vi "Dialog Tester - Preempt.vi"() -> ()   [LabVIEW 2021]
doc: "<b>TEST VI</b> checking the pre-empt action for pop up types"
uses:
  Standard/Input (DBL)/Input (DBL).lvclass
  Standard/Input (I32)/Input (I32).lvclass
  Standard/Input (String)/Input (String).lvclass
  Standard/Timeout/Timeout.lvclass
  Standard/Timeout One Button/Timeout One Button.lvclass
  Standard/Timeout Two Button/Timeout Two Button.lvclass
  Standard/Two Button/Two Button.lvclass
  Popup/Popup.lvclass
panel:
  out "Two-Button T.O. Choice? - val":bool
  out "Two-Button Choice? - val":bool
  out "Input Value (String - val)":string
  out "Input Value (I32 - val)":i32
  out "Input Value (DBL - close)":dbl
  out "Two-Button T.O. Choice? - close":bool
  out "Two-Button Choice? - close":bool
  out "Input Value (String - close)":string
  out "Input Value (I32 - close)":i32
  out "Input Value (DBL - val)":dbl
  out "iteration":i32
  in  "Error In":errorcluster
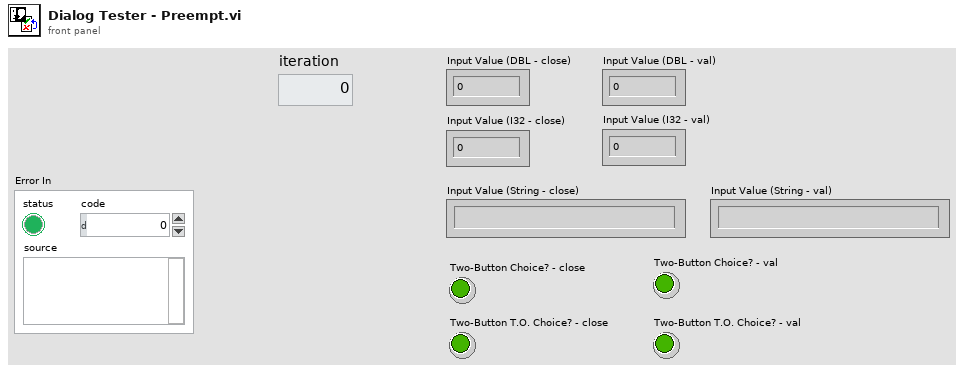
[diagram p1: front panel]
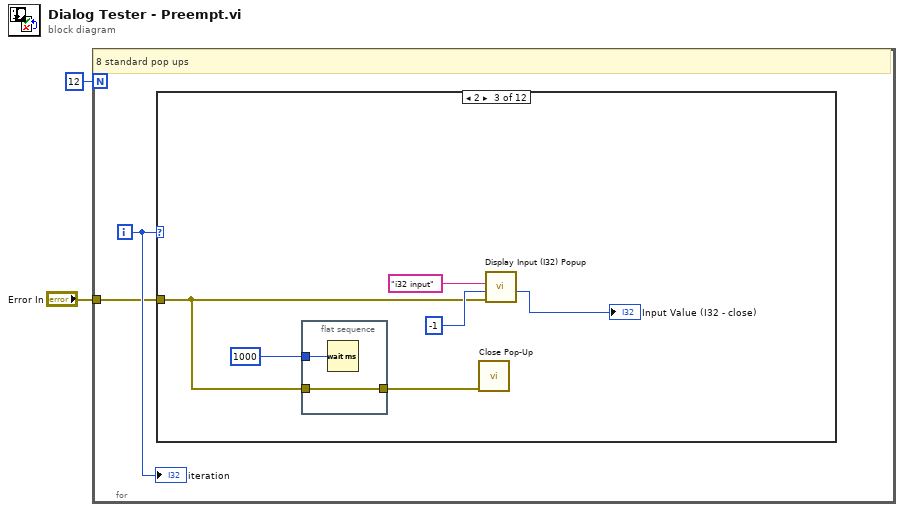
[diagram p0: block diagram]
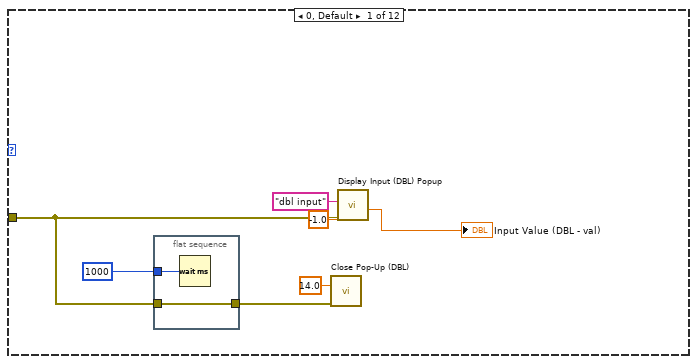
[diagram p2: hidden frame]
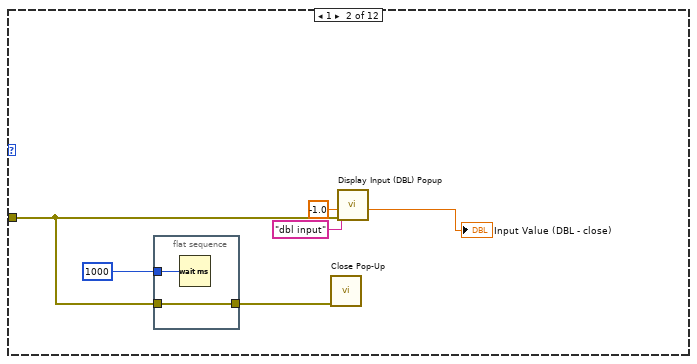
[diagram p3: hidden frame]
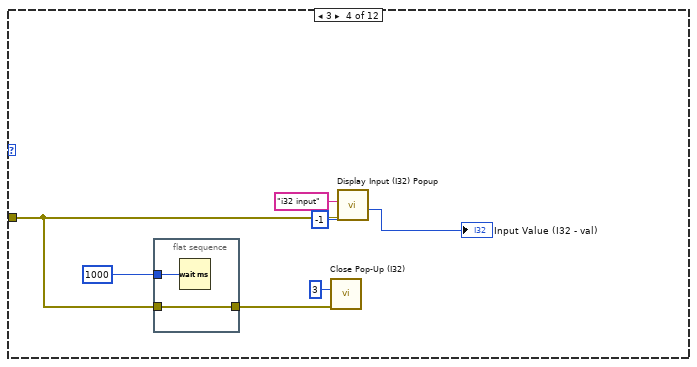
[diagram p4: hidden frame]
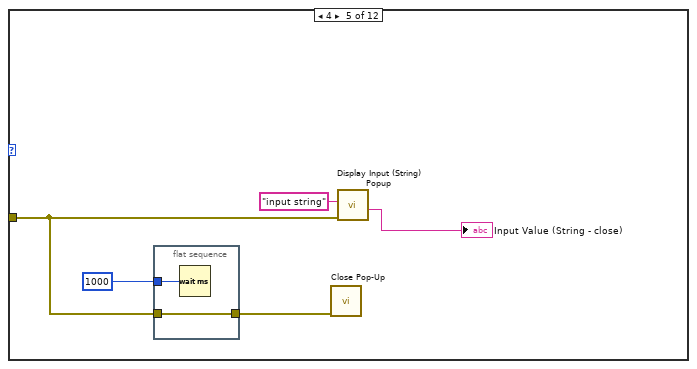
[diagram p5: hidden frame]
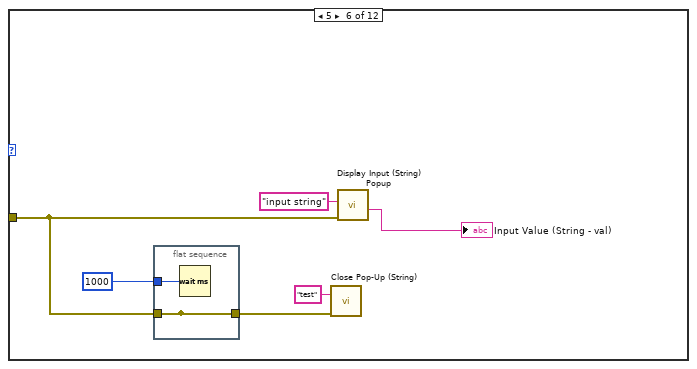
[diagram p6: hidden frame]
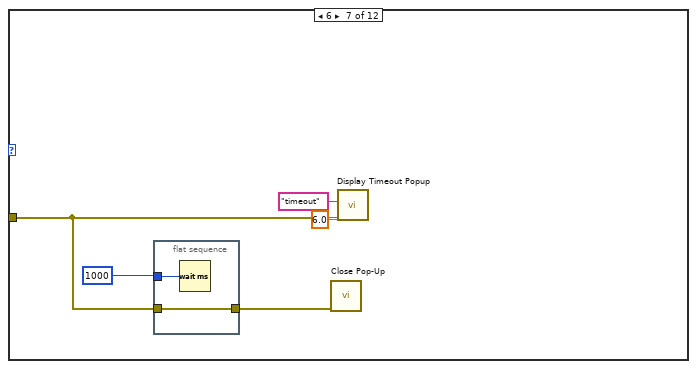
[diagram p7: hidden frame]
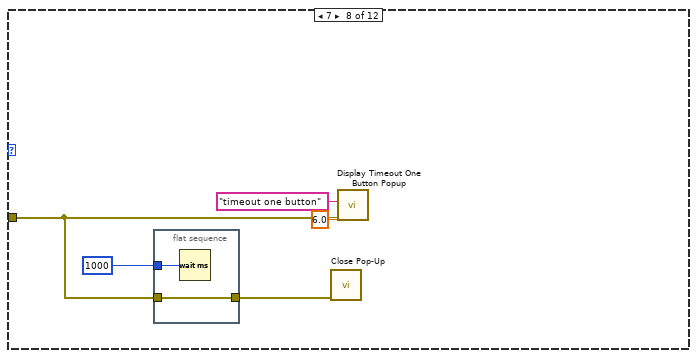
[diagram p8: hidden frame]
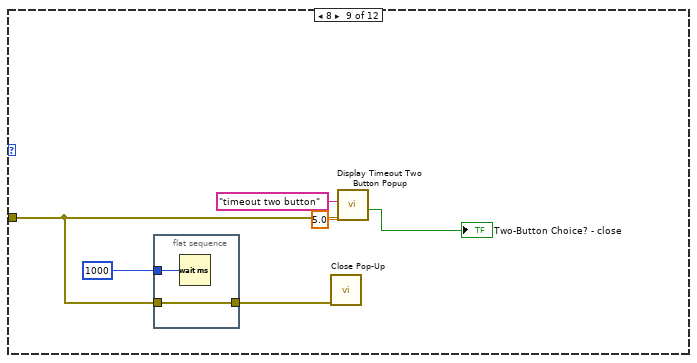
[diagram p9: hidden frame]
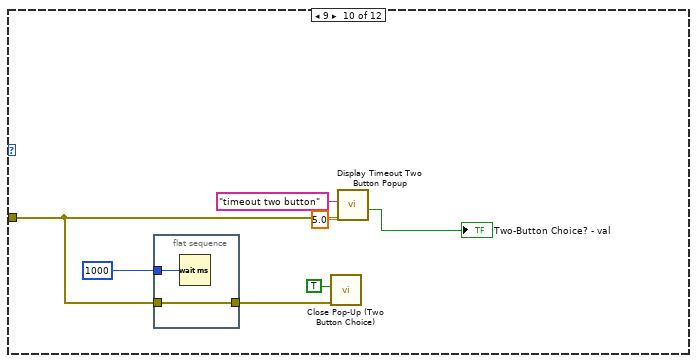
[diagram p10: hidden frame]
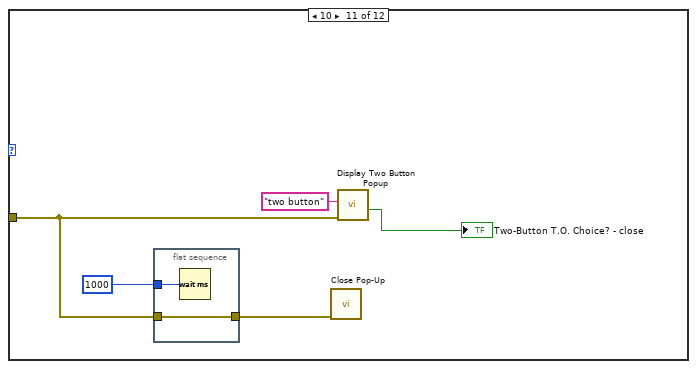
[diagram p11: hidden frame]
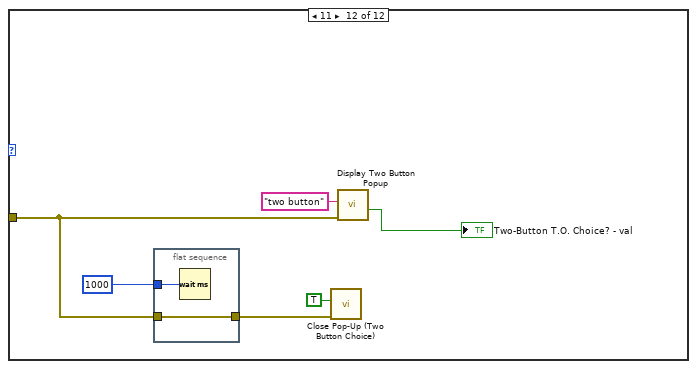
[diagram p12: hidden frame]
diagram:
  n1 = for {
    N: 12 -> [_]
    tunnel: "Error In" -> [w3]
    i -> [w4]
    # "8 standard pop ups"
    n2 = case shown="2" w4 {
      tunnel: w3 -> [w7 w16 w23 w31 w40 w47 w54 w62 w69 w77 w86 w93]
      frame 0, Default {
        n3 = flat-sequence {
          tunnel: u32 1000 ("milliseconds to wait") -> [w13]
          tunnel: [w12] -> w6
          tunnel: w7 -> [w12]
          frame #0 {
            n4 = Wait (ms)(milliseconds to wait=w13) -> ()  [unwired: 1 out]
          }
        }
        n5 = call "Close Pop-Up (DBL).vi"("error in"=w6, "DBL Default"=14.0) -> ()  [unwired: 9 in, 1 out]
        n6 = call "Display Input (DBL) Popup.vi"("error in"=w7, "Default Input"=-1.0, "Message"="dbl input") -> ("Input Value"=→"Input Value (DBL - val)":dbl)  [unwired: 7 in, 1 out]
      }
      frame 1 {
        n7 = flat-sequence {
          tunnel: u32 1000 ("milliseconds to wait") -> [w21]
          tunnel: [w20] -> w15
          tunnel: w16 -> [w20]
          frame #0 {
            n8 = Wait (ms)(milliseconds to wait=w21) -> ()  [unwired: 1 out]
          }
        }
        n9 = call "Close Pop-Up.vi"("error in"=w15) -> ()  [unwired: 10 in, 1 out]
        n10 = call "Display Input (DBL) Popup.vi"("error in"=w16, "Default Input"=-1.0, "Message"="dbl input") -> ("Input Value"=→"Input Value (DBL - close)":dbl)  [unwired: 7 in, 1 out]
      }
      frame 2 {
        n11 = flat-sequence {
          tunnel: u32 1000 ("milliseconds to wait") -> [w29]
          tunnel: [w28] -> w24
          tunnel: w23 -> [w28]
          frame #0 {
            n12 = Wait (ms)(milliseconds to wait=w29) -> ()  [unwired: 1 out]
          }
        }
        n13 = call "Close Pop-Up.vi"("error in"=w24) -> ()  [unwired: 10 in, 1 out]
        n14 = call "Display Input (I32) Popup.vi"("error in"=w23, "Default Input"=-1, "Message"="i32 input") -> ("Input Value"=→"Input Value (I32 - close)":i32)  [unwired: 7 in, 1 out]
      }
      frame 3 {
        n15 = flat-sequence {
          tunnel: u32 1000 ("milliseconds to wait") -> [w37]
          tunnel: [w36] -> _
          tunnel: w31 -> [w36]
          frame #0 {
            n16 = Wait (ms)(milliseconds to wait=w37) -> ()  [unwired: 1 out]
          }
        }
        n17 = call "Close Pop-Up (I32).vi"("error in"=w31, "I32 Default"=3) -> ()  [unwired: 9 in, 1 out]
        n18 = call "Display Input (I32) Popup.vi"("error in"=w31, "Default Input"=-1, "Message"="i32 input") -> ("Input Value"=→"Input Value (I32 - val)":i32)  [unwired: 7 in, 1 out]
      }
      frame 4 {
        n19 = flat-sequence {
          tunnel: u32 1000 ("milliseconds to wait") -> [w44]
          tunnel: [w43] -> w39
          tunnel: w40 -> [w43]
          frame #0 {
            n20 = Wait (ms)(milliseconds to wait=w44) -> ()  [unwired: 1 out]
          }
        }
        n21 = call "Close Pop-Up.vi"("error in"=w39) -> ()  [unwired: 10 in, 1 out]
        n22 = call "Display Input (String) Popup.vi"("error in"=w40, "Message"="input string") -> ("Input Value"=→"Input Value (String - close)":string)  [unwired: 8 in, 1 out]
      }
      frame 5 {
        n23 = flat-sequence {
          tunnel: u32 1000 ("milliseconds to wait") -> [w52]
          tunnel: [w51] -> w45
          tunnel: [w51] -> _
          tunnel: w47 -> [w51]
          frame #0 {
            n24 = Wait (ms)(milliseconds to wait=w52) -> ()  [unwired: 1 out]
          }
        }
        n25 = call "Close Pop-Up (String).vi"("error in"=w45, "String Default"="test") -> ()  [unwired: 9 in, 1 out]
        n26 = call "Display Input (String) Popup.vi"("error in"=w47, "Message"="input string") -> ("Input Value"=→"Input Value (String - val)":string)  [unwired: 8 in, 1 out]
      }
      frame 6 {
        n27 = flat-sequence {
          tunnel: u32 1000 ("milliseconds to wait") -> [w59]
          tunnel: [w58] -> w55
          tunnel: w54 -> [w58]
          frame #0 {
            n28 = Wait (ms)(milliseconds to wait=w59) -> ()  [unwired: 1 out]
          }
        }
        n29 = call "Close Pop-Up.vi"("error in"=w55) -> ()  [unwired: 10 in, 1 out]
        n30 = call "Display Timeout Popup.vi"("error in"=w54, "Timeout (s)"=6.0, "Message"="timeout") -> ()  [unwired: 7 in, 2 out]
      }
      frame 7 {
        n31 = flat-sequence {
          tunnel: u32 1000 ("milliseconds to wait") -> [w66]
          tunnel: [w65] -> w61
          tunnel: w62 -> [w65]
          frame #0 {
            n32 = Wait (ms)(milliseconds to wait=w66) -> ()  [unwired: 1 out]
          }
        }
        n33 = call "Close Pop-Up.vi"("error in"=w61) -> ()  [unwired: 10 in, 1 out]
        n34 = call "Display Timeout One Button Popup.vi"("error in"=w62, "Timeout (s)"=6.0, "Message"="timeout one button") -> ()  [unwired: 7 in, 2 out]
      }
      frame 8 {
        n35 = flat-sequence {
          tunnel: u32 1000 ("milliseconds to wait") -> [w74]
          tunnel: [w73] -> w68
          tunnel: w69 -> [w73]
          frame #0 {
            n36 = Wait (ms)(milliseconds to wait=w74) -> ()  [unwired: 1 out]
          }
        }
        n37 = call "Close Pop-Up.vi"("error in"=w68) -> ()  [unwired: 10 in, 1 out]
        n38 = call "Display Timeout Two Button Popup.vi"("error in"=w69, "Timeout (s)"=5.0, "Message"="timeout two button") -> ("Choice"=→"Two-Button Choice? - close":bool)  [unwired: 6 in, 2 out]
      }
      frame 9 {
        n39 = flat-sequence {
          tunnel: u32 1000 ("milliseconds to wait") -> [w83]
          tunnel: [w82] -> w76
          tunnel: w77 -> [w82]
          frame #0 {
            n40 = Wait (ms)(milliseconds to wait=w83) -> ()  [unwired: 1 out]
          }
        }
        n41 = call "Close Pop-Up (Two Button Choice).vi"("error in"=w76, "Two-Button Choice? (F)"=TRUE) -> ()  [unwired: 9 in, 1 out]
        n42 = call "Display Timeout Two Button Popup.vi"("error in"=w77, "Timeout (s)"=5.0, "Message"="timeout two button") -> ("Choice"=→"Two-Button Choice? - val":bool)  [unwired: 6 in, 2 out]
      }
      frame 10 {
        n43 = flat-sequence {
          tunnel: u32 1000 ("milliseconds to wait") -> [w90]
          tunnel: [w89] -> w85
          tunnel: w86 -> [w89]
          frame #0 {
            n44 = Wait (ms)(milliseconds to wait=w90) -> ()  [unwired: 1 out]
          }
        }
        n45 = call "Close Pop-Up.vi"("error in"=w85) -> ()  [unwired: 10 in, 1 out]
        n46 = call "Display Two Button Popup.vi"("error in"=w86, "Message"="two button") -> ("Choice"=→"Two-Button T.O. Choice? - close":bool)  [unwired: 8 in, 1 out]
      }
      frame 11 {
        n47 = flat-sequence {
          tunnel: u32 1000 ("milliseconds to wait") -> [w98]
          tunnel: [w97] -> w92
          tunnel: w93 -> [w97]
          frame #0 {
            n48 = Wait (ms)(milliseconds to wait=w98) -> ()  [unwired: 1 out]
          }
        }
        n49 = call "Close Pop-Up (Two Button Choice).vi"("error in"=w92, "Two-Button Choice? (F)"=TRUE) -> ()  [unwired: 9 in, 1 out]
        n50 = call "Display Two Button Popup.vi"("error in"=w93, "Message"="two button") -> ("Choice"=→"Two-Button T.O. Choice? - val":bool)  [unwired: 8 in, 1 out]
      }
    }
    "iteration" <- w4
  }
